vi "Perform Measurements.vi"(7 "error in":errorcluster, 8 "Measurement Context":refnum<class "Measure Call Context.lvclass">, 9 "Nominal output voltage":dbl, 10 "Reference values":T2) -> (0 "error out":errorcluster, 1 "Measurement Results":T1, 2 "Load out":refnum<k15>, 3 "Source out":refnum<k15>)   [LabVIEW 2021, in "Efficiency And Load Regulation_PMIC.lvlib"]
uses:
  Efficiency And Load Regulation_PMIC.lvlib
  Measurement Results.ctl
  <vilib>/Plug-In SDKs/Measurements/Measure Call Context/Measure Call Context.lvclass
  <vilib>/Plug-In SDKs/Measurements/Measure Call Context/Accessor/Is Canceled.vi
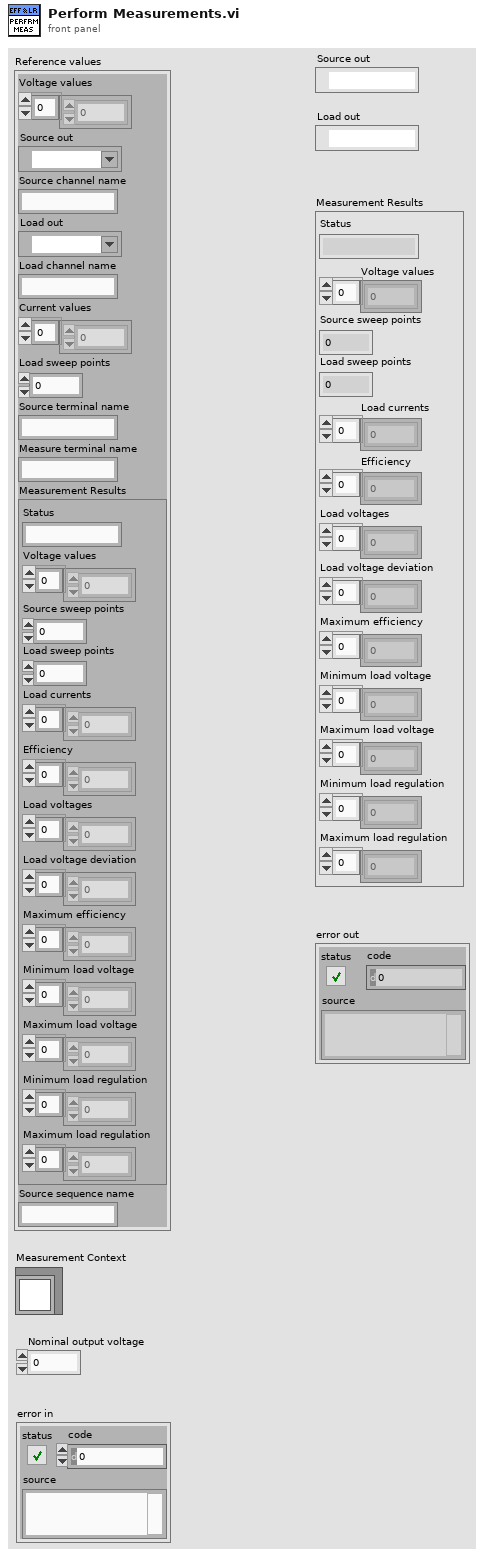
[diagram p1: front panel]
types:
  T1 = typedef "Efficiency And Load Regulation_PMIC.lvlib/Measurement Results.ctl" = cluster{"Status":string, "Voltage values":dbl[], "Source sweep points":i32, "Load sweep points":i32, "Load currents":dbl[], "Efficiency":dbl[], "Load voltages":dbl[], "Load voltage deviation":dbl[], "Maximum efficiency":dbl[], "Minimum load voltage":dbl[], "Maximum load voltage":dbl[], "Minimum load regulation":dbl[], "Maximum load regulation":dbl[]}
  T2 = cluster{"Voltage values":dbl[], "Source out":refnum<k15>, "Source channel name":string, "Load out":refnum<k15>, "Load channel name":string, "Current values":dbl[], "Load sweep points":i32, "Source terminal name":string, "Measure terminal name":string, "Measurement Results":T1, "Source sequence name":string}
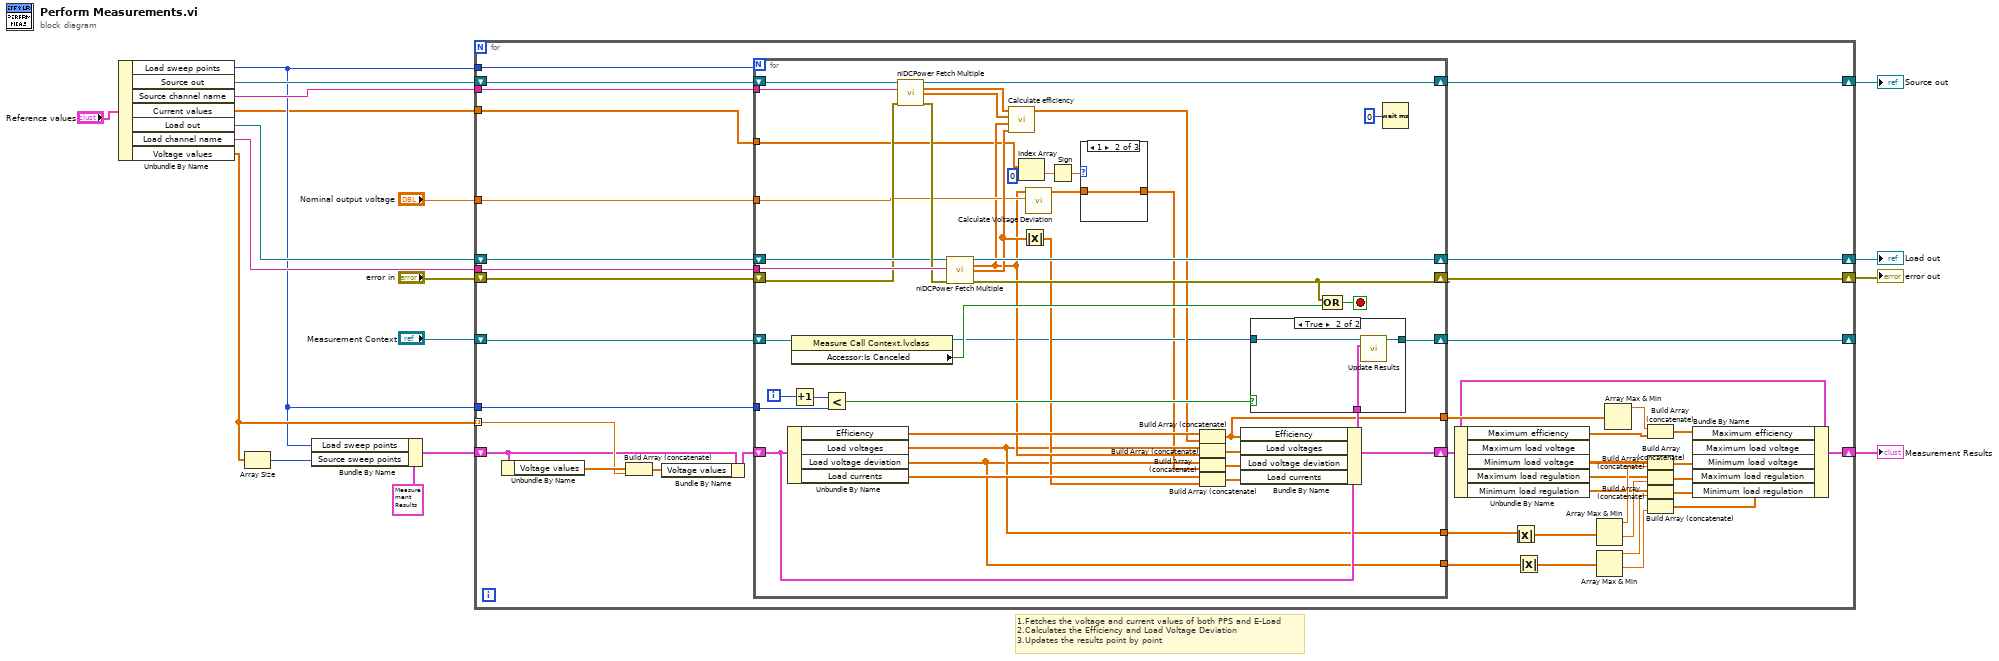
[diagram p0: block diagram]
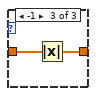
[diagram p3: hidden frame]
diagram:
  # "1.Fetches the voltage and current values of both PPS and E-Load\n2.Calculates the Efficiency and Load Voltage Deviation\n3.Updates the results point by point"
  n1 = Unbundle By Name("Reference values") -> ("Load sweep points"=w2:i32, "Source out"=w12:refnum<k15>, "Source channel name"=w11:string, "Current values"=w1:dbl[], "Load out"=w10:refnum<k15>, "Load channel name"=w9:string, "Voltage values"=w4:dbl[])
  n2 = Array Size(array=w4) -> (size(s)=w3:i32)
  n3 = Bundle By Name(cluster=T1 {"Status"="", "Voltage values"=[], "Source sweep points"=0, "Load sweep points"=0, "Load currents"=[], "Efficiency"=[], "Load voltages"=[], "Load voltage deviation"=[], "Maximum efficiency"=[], "Minimum load voltage"=[], "Maximum load voltage"=[], "Minimum load regulation"=[], "Maximum load regulation"=[]} ("Measurement Results"), "Load sweep points"=w2, "Source sweep points"=w3) -> (w7:T1)
  n4 = for {
    tunnel: "Nominal output voltage" -> [w55]
    tunnel: w11 -> [w53]
    tunnel: w9 -> [w51]
    tunnel: w2 -> [w50]
    shift-right: [w58] -> w17
    shift-left: "error in" -> [w59]
    shift-right: [w56] -> w15
    shift-left: w12 -> [w54]
    shift-right: [w57] -> w16
    shift-left: w10 -> [w52]
    shift-right: [w48] -> _
    shift-left: "Measurement Context" -> [w49]
    shift-right: [w41] -> w6
    shift-left: w7 -> [w44]
    tunnel: w4 -> [w45] mode=indexing
    tunnel: w2 -> [w47]
    tunnel: w1 -> [w19]
    n5 = Unbundle By Name(w44) -> ("Voltage values"=w46:dbl[])
    n6 = Build Array (concatenate)(w46, w45) -> (w42:dbl[])
    n7 = Bundle By Name(cluster=w44, "Voltage values"=w42) -> (w43:T1)
    n8 = for {
      N: w50 -> [_]
      tunnel: w51 -> [w98]
      tunnel: w53 -> [w97]
      shift-right: [w99] -> w57
      shift-left: w52 -> [w95]
      shift-right: [w88] -> w58
      shift-left: w59 -> [w94]
      shift-right: [w100] -> w56
      shift-left: w54 -> [w101]
      tunnel: w55 -> [w90]
      shift-right: [w71] -> w48
      shift-left: w49 -> [w84]
      shift-right: [w74] -> w24
      shift-left: w43 -> [w75]
      tunnel: w47 -> [w70]
      tunnel: [w68] -> w40
      tunnel: [w67] -> w22
      tunnel: [w66] -> w23
      tunnel: w19 -> [w63]
      i -> [w86]
      stop <- w73 stop-if-true
      n9 = Unbundle By Name(w75) -> ("Efficiency"=w79:dbl[], "Load voltages"=w67:dbl[], "Load voltage deviation"=w66:dbl[], "Load currents"=w80:dbl[])
      n10 = property class="Measure Call Context.lvclass"(reference=w84) -> (reference out=w72:refnum<class "Measure Call Context.lvclass">, "Accessor:Is Canceled"=w89:bool)  [unwired: 1 in, 1 out]
      n11 = Increment(x=w86) -> (x+1=w87:i32)
      n12 = Less?(x=w87, y=w70) -> (x < y?=w85:bool)
      n13 = call <instrlib>:"niDCPower Fetch Multiple.vi"("instrument handle"=w101, "channel name"=w97, "error in (no error)"=w94) -> ("instrument handle out"=w100:refnum<k15>, "voltage measurements"=w93:dbl[], "current measurements"=w92:dbl[], "error out"=w96:errorcluster)  [unwired: 2 in, 7 out]
      n14 = call <instrlib>:"niDCPower Fetch Multiple.vi"("instrument handle"=w95, "channel name"=w98, "error in (no error)"=w96) -> ("instrument handle out"=w99:refnum<k15>, "voltage measurements"=w77:dbl[], "current measurements"=w91:dbl[], "error out"=w88:errorcluster)  [unwired: 2 in, 7 out]
      n15 = call "Calculate efficiency.vi"("load current measurements"=w91, "load voltage measurements"=w77, "source current measurements"=w92, "source voltage measurements"=w93) -> ("Efficiency(%)"=w78:dbl[])  [unwired: 7 in]
      n16 = Index Array(array=w63, index=0) -> (element=w64:dbl)
      n17 = Absolute Value(x=w91) -> (abs(x)=w76:dbl[])
      n18 = call "Calculate Voltage Deviation.vi"("Nominal output voltage"=w90, "Voltage measurements"=w77) -> ("Load voltage deviation"=w60:dbl[])  [unwired: 9 in]
      n19 = Sign(1:w64) -> (0:w62:dbl)
      n20 = case shown="1" w62 {
        tunnel: [w102 w103 w105] -> w65
        tunnel: w60 -> [w102 w103 w104]
        frame 0, Default {
        }
        frame 1 {
        }
        frame -1 {
          n21 = Absolute Value(x=w104) -> (abs(x)=w105:dbl[])
        }
      }
      n22 = Build Array (concatenate)(w79, w78) -> (w68:dbl[])
      n23 = Build Array (concatenate)(w67, w77) -> (w81:dbl[])
      n24 = Build Array (concatenate)(w66, w65) -> (w82:dbl[])
      n25 = Build Array (concatenate)(w80, w76) -> (w83:dbl[])
      n26 = Bundle By Name(cluster=w75, "Efficiency"=w68, "Load voltages"=w81, "Load voltage deviation"=w82, "Load currents"=w83) -> (w74:T1)
      n27 = case shown="True" w85 {
        tunnel: w74 -> [_ w109]
        tunnel: w72 -> [w106 w108]
        tunnel: [w106 w107] -> w71
        frame False {
        }
        frame True {
          n28 = call <vilib>:"Update Results.vi"("measurement results"=w109, "measure call context in"=w108) -> ("measure call context out"=w107:refnum<class "Measure Call Context.lvclass">)  [unwired: 8 in, 1 out]
        }
      }
      n29 = Compound Arithmetic op=OR(w88, w89) -> (w73:bool)
      n30 = Wait (ms)(milliseconds to wait=u32 0) -> ()  [unwired: 1 out]
    }
    n31 = Unbundle By Name(w24) -> ("Maximum efficiency"=w38:dbl[], "Maximum load voltage"=w37:dbl[], "Minimum load voltage"=w35:dbl[], "Maximum load regulation"=w33:dbl[], "Minimum load regulation"=w32:dbl[])
    n32 = Absolute Value(x=w22) -> (abs(x)=w21:dbl[])
    n33 = Absolute Value(x=w23) -> (abs(x)=w20:dbl[])
    n34 = Array Max & Min(array=w21) -> (max value=w36:dbl, min value=w34:dbl)  [unwired: 2 out]
    n35 = Array Max & Min(array=w20) -> (max value=w31:dbl, min value=w30:dbl)  [unwired: 2 out]
    n36 = Array Max & Min(array=w40) -> (max value=w39:dbl)  [unwired: 3 out]
    n37 = Build Array (concatenate)(w39, w38) -> (w29:dbl[])
    n38 = Build Array (concatenate)(w37, w36) -> (w28:dbl[])
    n39 = Build Array (concatenate)(w35, w34) -> (w27:dbl[])
    n40 = Build Array (concatenate)(w33, w31) -> (w26:dbl[])
    n41 = Build Array (concatenate)(w32, w30) -> (w25:dbl[])
    n42 = Bundle By Name(cluster=w24, "Maximum efficiency"=w29, "Maximum load voltage"=w28, "Minimum load voltage"=w27, "Maximum load regulation"=w26, "Minimum load regulation"=w25) -> (w41:T1)
  }
  "error out" <- w17
  "Load out" <- w16
  "Source out" <- w15
  "Measurement Results" <- w6
